vi "Measurement Logic.vi"(8 "error in":errorcluster, 9 "measurement configuration":T2, 10 "measure call context in":refnum<class "Measure Call Context.lvclass">, 11 "Stop OOB Server UE":refnum<user-event>) -> (0 "error out":errorcluster, 1 "measurement results":T1 {"Scanned Addresses" format="%.0x"}, 2 "measure call context out":refnum<class "Measure Call Context.lvclass">)   [LabVIEW 2025, in "I2C Bus Monitor.lvclass"]
doc: "Contains the core logic for executing the measurement."
uses:
  I2C Bus Monitor.lvclass
  <vilib>/Plug-In SDKs/Measurements/Measure Call Context/Measure Call Context.lvclass
  Measurement Configuration.ctl
  Measurement Results.ctl
  Typedefs/Logic Data.ctl
  Typedefs/State.ctl
  <instrlib>/FlexRIO/CSI-2/v2/FPGA/Types/Timestamp ID.ctl
  SubVIs/I2C Message Buffer - Create.vi
  SubVIs/I2C Message Buffer - Enqueue.vi
  SubVIs/I2C Message Buffer - Check.vi
  SubVIs/Error Global.vi
  SubVIs/I2C Message Buffer - Destroy.vi
  I2C Bus Monitor.lvclass/I2C Bus Monitor.ctl
  OOB Data Transfer/OOB Data Transfer.lvlib
  <instrlib>/_niInstr/Basic Elements/v1/FPGA/niInstr Basic Elements v1 FPGA.lvlib
  <instrlib>/FlexRIO/CSI-2/v2/FPGA/NI CSI-2 API FPGA v2.lvlib
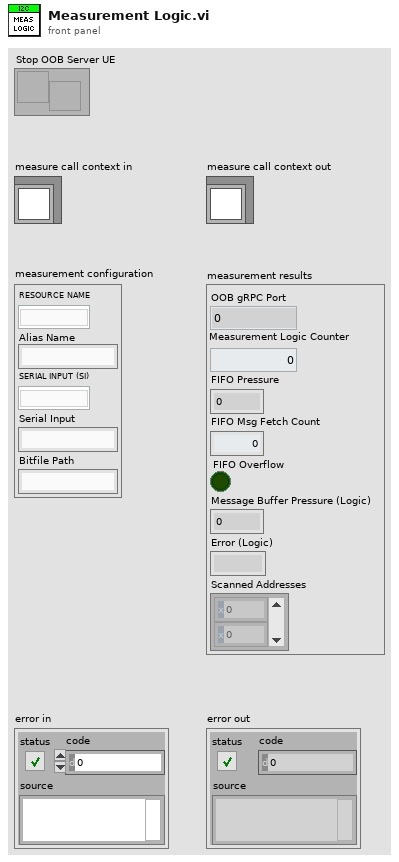
[diagram p1: front panel]
types:
  T1 = typedef "I2C Bus Monitor.lvclass/Measurement Results.ctl" = cluster{"OOB gRPC Port":i32, "Measurement Logic Counter":i32, "FIFO Pressure":u32, "FIFO Msg Fetch Count":i32, "FIFO Overflow":bool, "Message Buffer Pressure (Logic)":i32, "Error (Logic)":string, "Scanned Addresses":i32[]}
  T2 = typedef "I2C Bus Monitor.lvclass/Measurement Configuration.ctl" = cluster{"RESOURCE NAME":u32, "Alias Name":string, "SERIAL INPUT (SI)":u32, "Serial Input":string, "Bitfile Path":string}
  T3 = typedef "I2C Bus Monitor.lvclass/Logic Data.ctl" = cluster{"State":T4, "FPGA Ref":refnum<k20>, "Timestamp ID":T5, "Results":T1}
  T4 = typedef "I2C Bus Monitor.lvclass/State.ctl" = enum16{"Init", "Execute", "Results", "Error", "Close"}
  T5 = typedef "NI CSI-2 API FPGA v2.lvlib/Timestamp ID.ctl" = enum8{"SI0 LLP", "SI1 LLP", "SI2 LLP", "SI3 LLP", "SI4 LLP", "SI5 LLP", "SI6 LLP", "SI7 LLP", "SO0 LLP", "SO1 LLP", "SO2 LLP", "SO3 LLP", "SO4 LLP", "SO5 LLP", "SO6 LLP", "SO7 LLP", "Ser0 GPIO Bank", "Ser1 GPIO Bank", "Ser2 GPIO Bank", "Ser3 GPIO Bank", "Ser4 GPIO Bank", "Ser5 GPIO Bank", "Ser6 GPIO Bank", "Ser7 GPIO Bank", "Des0 GPIO Bank", "Des1 GPIO Bank", "Des2 GPIO Bank", "Des3 GPIO Bank", "Des4 GPIO Bank", "Des5 GPIO Bank", "Des6 GPIO Bank", "Des7 GPIO Bank", "User0", "User1", "User2", "User3", "User4", "User5", "User6", "User7", "User8", "User9", "User10", "User11", "User12", "User13", "User14", "User15", "User16", "User17", "User18", "User19", "User20", "User21", "User22", "User23", "User24", "User25", "User26", "User27", "User28", "User29", "User30", "User31"}
  T6 = typedef "OOB Data Transfer.lvlib/OOB to Logic Data.ctl" = cluster{"PauseResume":bool, "Export":string, "Scan Bus":bool, "I2C Script":cluster{"Send":bool, "Path":string, "Complex":bool}, "I2C CMD":cluster{"Send":bool, "SLAVE ADDR.":u8, "REG. ADDR.":u16, "DATA":u8, "R/W":bool}}
  T7 = cluster{"Send":bool, "SLAVE ADDR.":u8, "REG. ADDR.":u16, "DATA":u8, "R/W":bool}
  T8 = cluster{"Serial Input":string, "SLAVE ADDR.":u8, "REG. ADDR.":u16, "DATA":u8, "R/W":bool}
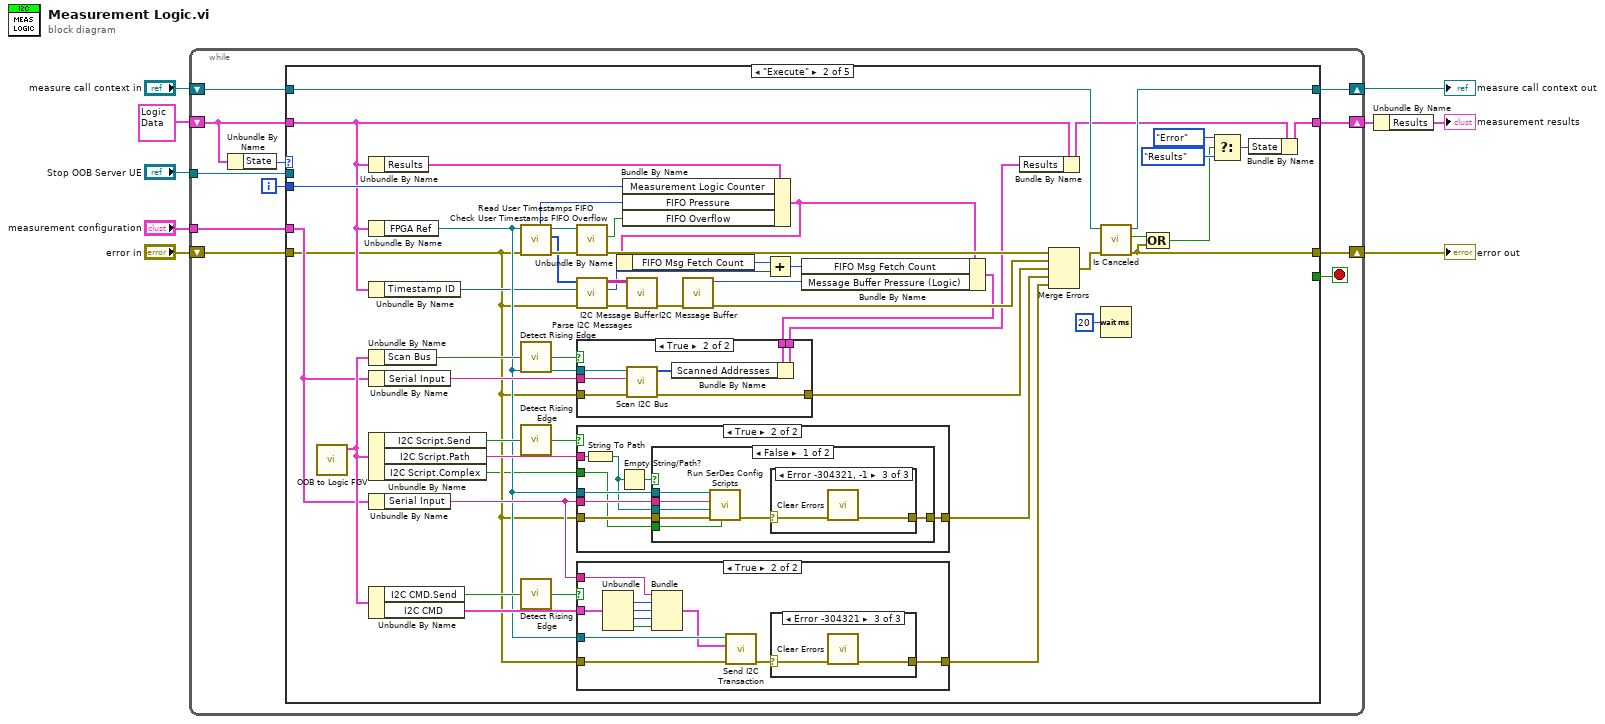
[diagram p0: block diagram]
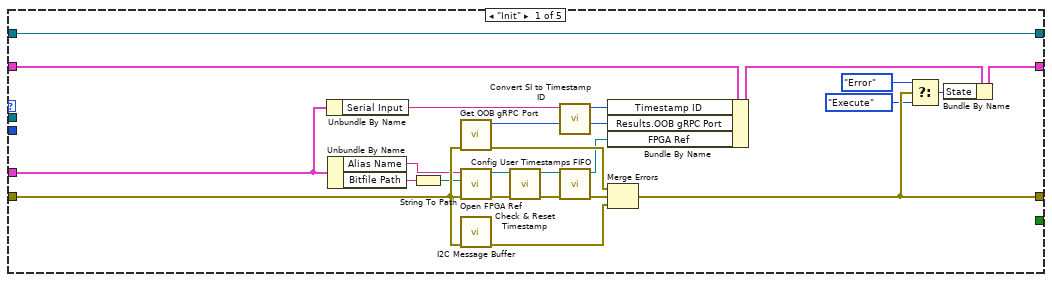
[diagram p2: hidden frame]
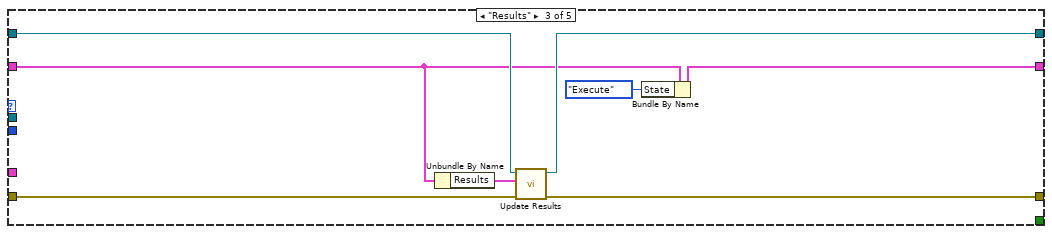
[diagram p11: hidden frame]
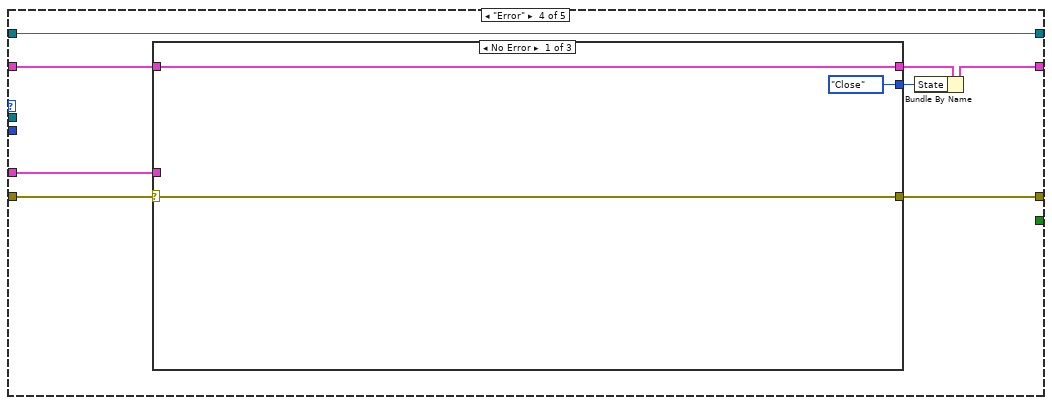
[diagram p12: hidden frame]
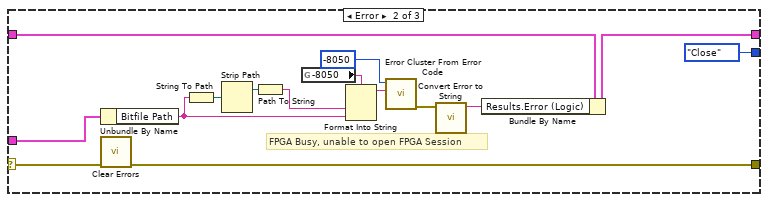
[diagram p13: hidden frame]
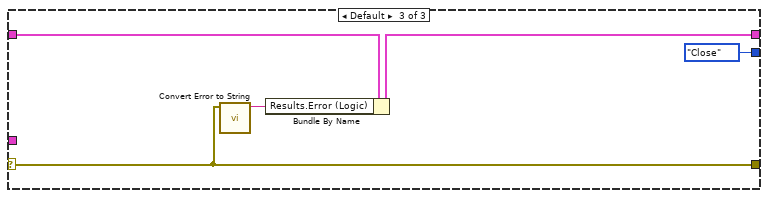
[diagram p14: hidden frame]
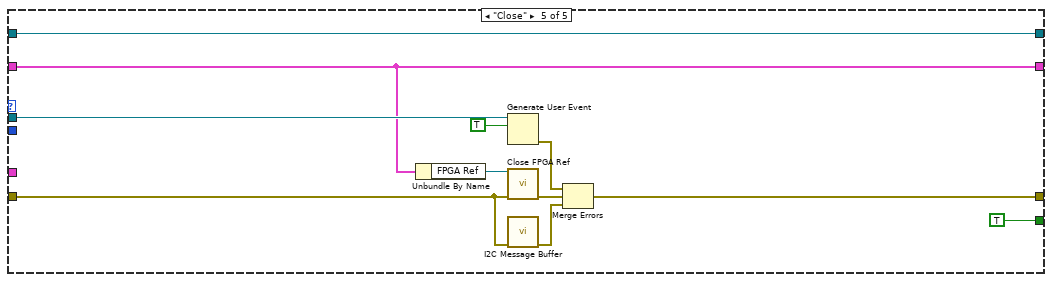
[diagram p15: hidden frame]
diagram:
  n1 = while {
    shift-right: [w15] -> w2
    shift-left: T3 {"State"=enum."Init", "FPGA Ref"=refnum, "Timestamp ID"=enum."SI0 LLP", "Results"={"OOB gRPC Port"=0, "Measurement Logic Counter"=0, "FIFO Pressure"=0, "FIFO Msg Fetch Count"=0, "FIFO Overflow"=FALSE, "Message Buffer Pressure (Logic)"=0, "Error (Logic)"="", "Scanned Addresses"=[]}} -> [w14]
    shift-right: [w10] -> w3
    shift-left: "error in" -> [w20]
    tunnel: "Stop OOB Server UE" -> [w18]
    tunnel: "measurement configuration" -> [w16]
    shift-right: [w11] -> w5
    shift-left: "measure call context in" -> [w17]
    i -> [w12]
    stop <- w19 stop-if-true
    n2 = Unbundle By Name(w14) -> ("State"=w13:T4)
    n3 = case shown="\"Execute\"" w13 {
      tunnel: w20 -> [w43 w49 w147 w156 w185]
      tunnel: [_ _ _ _ TRUE] -> w19
      tunnel: w18 -> [_ _ _ _ w189]
      tunnel: w17 -> [w28 w82 w145 w150 w190]
      tunnel: w16 -> [w31 w73 _ w151 _]
      tunnel: w14 -> [w42 w51 w143 w157 w181]
      tunnel: [w24 w84 w149 w153 w181] -> w15
      tunnel: w12 -> [_ w71 _ _ _]
      tunnel: [w22 w75 w146 w155 w184] -> w10
      tunnel: [w28 w81 w144 w150 w190] -> w11
      frame "Init" {
        n4 = Unbundle By Name(w31) -> ("Serial Input"=w41:string)
        n5 = Unbundle By Name(w31) -> ("Alias Name"=w36:string, "Bitfile Path"=w37:string)
        n6 = String To Path(string=w37) -> (path=w38:path)
        n7 = call "Get OOB gRPC Port.vi"("error in (no error)"=w43) -> ("error out"=w44:errorcluster, "OOB gRPC Port"=w27:i32)  [unwired: 9 in]
        n8 = call "Open FPGA Ref.vi"("error in (no error)"=w43, "Bitfile Path"=w38, "Device address"=w36) -> ("error out"=w39:errorcluster, "FPGA Ref out"=w34:refnum<k20>)  [unwired: 7 in]
        n9 = call-poly "I2C Message Buffer.vi"("error in (no error)"=w43) -> ("error out"=w32:errorcluster)  [unwired: 10 in]
        n10 = call "Check & Reset Timestamp.vi"("error in (no error)"=w39, "FPGA Ref in"=w34) -> ("error out"=w40:errorcluster, "FPGA Ref out"=w35:refnum<k20>)  [unwired: 8 in]
        n11 = call "Convert SI to Timestamp ID.vi"("SI Channel"=w41) -> ("Timestamp ID"=w29:T5)  [unwired: 10 in]
        n12 = call "Config User Timestamps FIFO.vi"("error in (no error)"=w40, "FPGA Ref in"=w35) -> ("error out"=w33:errorcluster, "FPGA Ref out"=w30:refnum<k20>)  [unwired: 8 in]
        n13 = Bundle By Name(cluster=w42, "Timestamp ID"=w29, "Results.OOB gRPC Port"=w27, "FPGA Ref"=w30) -> (w25:T3)
        n14 = Merge Errors(w44, w33, w32) -> (w22:errorcluster)
        n15 = Select(t=State."Error", s=w22, f=State."Execute") -> (s? t:f=w23:T4)
        n16 = Bundle By Name(cluster=w25, "State"=w23) -> (w24:T3)
      }
      frame "Execute" {
        n17 = call "OOB to Logic FGV.vi"() -> ("OOB to Logic Data out"=w88:T6)  [unwired: 10 in, 1 out]
        n18 = Unbundle By Name(w51) -> ("Results"=w52:T1)
        n19 = Unbundle By Name(w51) -> ("FPGA Ref"=w65:refnum<k20>)
        n20 = Unbundle By Name(w51) -> ("Timestamp ID"=w58:T5)
        n21 = Unbundle By Name(w88) -> ("Scan Bus"=w66:bool)
        n22 = Unbundle By Name(w73) -> ("Serial Input"=w67:string)
        n23 = Unbundle By Name(w88) -> ("I2C Script.Send"=w93:bool, "I2C Script.Path"=w92:string, "I2C Script.Complex"=w45:bool)
        n24 = Unbundle By Name(w73) -> ("Serial Input"=w80:string)
        n25 = Unbundle By Name(w88) -> ("I2C CMD.Send"=w90:bool, "I2C CMD"=w87:T7)
        n26 = call "Read User Timestamps FIFO.vi"("error in (no error)"=w49, "FPGA Ref in"=w65) -> ("error out"=w95:errorcluster, "Data"=w59:u64[], "FPGA Ref out"=w86:refnum<k20>, "Elements Remaining"=w70:u32)  [unwired: 6 in]
        n27 = call <instrlib>:"Detect Rising Edge.vi"("signal"=w66) -> ("edge detected"=w56:bool)  [unwired: 14 in]
        n28 = call <instrlib>:"Detect Rising Edge.vi"("signal"=w93) -> ("edge detected"=w91:bool)  [unwired: 14 in]
        n29 = call <instrlib>:"Detect Rising Edge.vi"("signal"=w90) -> ("edge detected"=w89:bool)  [unwired: 14 in]
        n30 = call "Check User Timestamps FIFO Overflow.vi"("error in (no error)"=w95, "FPGA Ref in"=w86) -> ("error out"=w85:errorcluster, "User Timestamp FIFO Overflow"=w69:bool)  [unwired: 7 in, 1 out]
        n31 = call "Parse I2C Messages.vi"("error in (no error)"=w49, "Timestamp ID"=w58, "User Timestamps"=w59) -> ("error out"=w61:errorcluster, "Count"=w55:i32, "I2C Messages"=w60:string[][])  [unwired: 6 in]
        n32 = case shown="True" w91 {
          tunnel: w92 -> [_ w128]
          tunnel: w49 -> [w121 w127]
          tunnel: w65 -> [_ w129]
          tunnel: w80 -> [_ w126]
          tunnel: [w121 w125] -> w68
          tunnel: w45 -> [_ w122]
          frame False {
          }
          frame True {
            n33 = String To Path(string=w128) -> (path=w123:path)
            n34 = Empty String/Path?(string/path=w123) -> (empty?=w124:bool)
            n35 = case shown="False" w124 {
              tunnel: w129 -> [w135 _]
              tunnel: w123 -> [w134 _]
              tunnel: w127 -> [w136 w141]
              tunnel: w126 -> [w131 _]
              tunnel: [w132 w141] -> w125
              tunnel: w122 -> [w130 _]
              frame False {
                n36 = call "Run SerDes Config Scripts.vi"("Complex Serdes Scripts"=w130, "error in (no error)"=w136, "configuration scripts"=w134, "serial channels"=w131, "FPGA Ref In"=w135) -> ("error out"=w133:errorcluster)  [unwired: 4 in, 2 out]
                n37 = case shown="Error -304321, -1" w133 {
                  selector: w133 -> [w137 w138 w140]
                  tunnel: [w137 w138 w139] -> w132
                  frame No Error {
                  }
                  frame Default {
                  }
                  frame Error {
                    n38 = call <vilib>:"Clear Errors.vi"("error in (no error)"=w140) -> ("error out"=w139:errorcluster)  [unwired: 5 in, 1 out]
                  }
                }
              }
              frame True {
              }
            }
          }
        }
        n39 = case shown="True" w89 {
          tunnel: w87 -> [_ w114]
          tunnel: w49 -> [w105 w115]
          tunnel: w65 -> [_ w116]
          tunnel: [w105 w106] -> w74
          tunnel: w80 -> [_ w109]
          frame False {
          }
          frame True {
            n40 = Unbundle(w114) -> ("SLAVE ADDR."=w113:u8, "REG. ADDR."=w112:u16, "DATA"=w111:u8, "R/W"=w110:bool)  [unwired: 1 out]
            n41 = Bundle("Serial Input"=w109, "SLAVE ADDR."=w113, "REG. ADDR."=w112, "DATA"=w111, "R/W"=w110) -> (w108:T8)  [unwired: 1 in]
            n42 = call "Send I2C Transaction.vi"("Error In"=w115, "I2C Command"=w108, "FPGA Ref in"=w116) -> ("Error Out"=w107:errorcluster)  [unwired: 6 in, 2 out]
            n43 = case shown="Error -304321" w107 {
              selector: w107 -> [w117 w118 w120]
              tunnel: [w117 w118 w119] -> w106
              frame No Error {
              }
              frame Default {
              }
              frame Error {
                n44 = call <vilib>:"Clear Errors.vi"("error in (no error)"=w120) -> ("error out"=w119:errorcluster)  [unwired: 5 in, 1 out]
              }
            }
          }
        }
        n45 = Bundle By Name(cluster=w52, "Measurement Logic Counter"=w71, "FIFO Pressure"=w70, "FIFO Overflow"=w69) -> (w50:T1)
        n46 = Unbundle By Name(w50) -> ("FIFO Msg Fetch Count"=w53:i32)
        n47 = call-poly "I2C Message Buffer.vi"("error in (no error)"=w61, "I2C Messages"=w60) -> ("error out"=w62:errorcluster)  [unwired: 9 in]
        n48 = call-poly "I2C Message Buffer.vi"("error in (no error)"=w62) -> ("error out"=w57:errorcluster, "Transactions"=w63:i32)  [unwired: 8 in, 1 out]
        n49 = Add(x=w53, y=w55) -> (x+y=w54:i32)
        n50 = Bundle By Name(cluster=w50, "FIFO Msg Fetch Count"=w54, "Message Buffer Pressure (Logic)"=w63) -> (w48:T1)
        n51 = case shown="True" w56 {
          tunnel: w67 -> [_ w104]
          tunnel: w65 -> [_ w103]
          tunnel: w49 -> [w96 w101]
          tunnel: w48 -> [w97 w100]
          tunnel: [w97 w99] -> w47
          tunnel: [w96 w98] -> w46
          frame False {
          }
          frame True {
            n52 = call "Scan I2C Bus.vi"("error in (no error)"=w101, "Serial Input"=w104, "FPGA Ref"=w103) -> ("error out"=w98:errorcluster, "Scanned Addresses"=w102:i32[])  [unwired: 7 in]
            n53 = Bundle By Name(cluster=w100, "Scanned Addresses"=w102) -> (w99:T1)
          }
        }
        n54 = Bundle By Name(cluster=w51, "Results"=w47) -> (w72:T3)
        n55 = Merge Errors(w85, w57, w46, w68, w74) -> (w76:errorcluster)
        n56 = call <vilib>:"Is Canceled.vi"("error in"=w76, "measure call context in"=w82) -> ("error out"=w75:errorcluster, "is canceled?"=w94:bool, "measure call context out"=w81:refnum<class "Measure Call Context.lvclass">)  [unwired: 7 in]
        n57 = Wait (ms)(milliseconds to wait=u32 20) -> ()  [unwired: 1 out]
        n58 = Compound Arithmetic op=OR(w94, w75) -> (w77:bool)
        n59 = Select(t=State."Error" ("State"), s=w77, f=State."Results") -> (s? t:f=w79:T4)
        n60 = Bundle By Name(cluster=w72, "State"=w79) -> (w84:T3)
      }
      frame "Results" {
        n61 = Unbundle By Name(w143) -> ("Results"=w142:T1)
        n62 = call <vilib>:"Update Results.vi"("error in"=w147, "measurement results"=w142, "measure call context in"=w145) -> ("error out"=w146:errorcluster, "measure call context out"=w144:refnum<class "Measure Call Context.lvclass">)  [unwired: 7 in]
        n63 = Bundle By Name(cluster=w143, "State"=State."Execute") -> (w149:T3)
      }
      frame "Error" {
        n64 = case shown="No Error" w156 {
          selector: w156 -> [w159 w172 w176]
          tunnel: w157 -> [w160 w167 w177]
          tunnel: [w160 w174 w179] -> w152
          tunnel: [w159 w171 w176] -> w155
          tunnel: [State."Close" ("State") State."Close" ("State") State."Close" ("State")] -> w154
          tunnel: w151 -> [_ w166 _]
          frame No Error {
          }
          frame Error {
            # "FPGA Busy, unable to open FPGA Session"
            n65 = Unbundle By Name(w166) -> ("Bitfile Path"=w162:string)
            n66 = call <vilib>:"Clear Errors.vi"("error in (no error)"=w172) -> ("error out"=w171:errorcluster)  [unwired: 5 in, 1 out]
            n67 = String To Path(string=w162) -> (path=w164:path)
            n68 = Strip Path(path=w164) -> (stripped path=w163:path)  [unwired: 1 out]
            n69 = Path To String(path=w163) -> (string=w161:string)
            n70 = global read "Error Global.vi" "-8050"() -> (w170:string)
            n71 = Format Into String(format string=w170, w161, w162) -> (resulting string=w169:string)  [unwired: 2 in, 1 out]
            n72 = call <vilib>:"Error Cluster From Error Code.vi"("error message (\"\")"=w169, "error code (0)"=-8050) -> ("error out"=w165:errorcluster)  [unwired: 7 in]
            n73 = call "Convert Error to String.vi"("error in (no error)"=w165) -> ("Error (Logic)"=w173:string)  [unwired: 10 in]
            n74 = Bundle By Name(cluster=w167, "Results.Error (Logic)"=w173) -> (w174:T3)
          }
          frame Default {
            n75 = call "Convert Error to String.vi"("error in (no error)"=w176) -> ("Error (Logic)"=w178:string)  [unwired: 10 in]
            n76 = Bundle By Name(cluster=w177, "Results.Error (Logic)"=w178) -> (w179:T3)
          }
        }
        n77 = Bundle By Name(cluster=w152, "State"=w154) -> (w153:T3)
      }
      frame "Close" {
        n78 = Unbundle By Name(w181) -> ("FPGA Ref"=w183:refnum<k20>)
        n79 = Generate User Event(user event=w189, event data cluster=TRUE ("event data")) -> (error out=w182:errorcluster)  [unwired: 2 in, 1 out]
        n80 = call "Close FPGA Ref.vi"("error in (no error)"=w185, "FPGA Ref in"=w183) -> ("error out"=w186:errorcluster)  [unwired: 9 in]
        n81 = call-poly "I2C Message Buffer.vi"("error in (no error)"=w185) -> ("error out"=w187:errorcluster)  [unwired: 10 in]
        n82 = Merge Errors(w182, w186, w187) -> (w184:errorcluster)
      }
    }
  }
  "error out" <- w3
  "measure call context out" <- w5
  n83 = Unbundle By Name(w2) -> ("Results"=→"measurement results":T1)
